vi "Day 11.vi"() -> ()   [LabVIEW 2021]
uses:
  <vilib>/Utility/file.llb/Read Delimited Spreadsheet (string).vi
panel:
  out "Input":i32[][](array[numeric])
  out "Part 2":i32
  out "Part 1":i32
  in  "Input File":enum32{"example input", "input"}(radio)
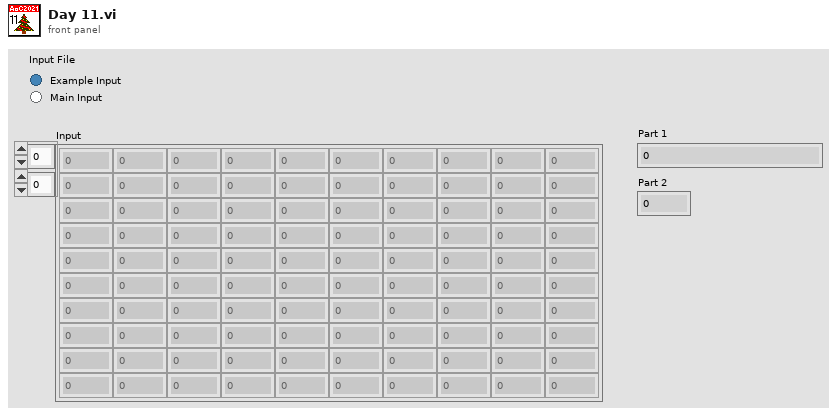
[diagram p1: front panel]
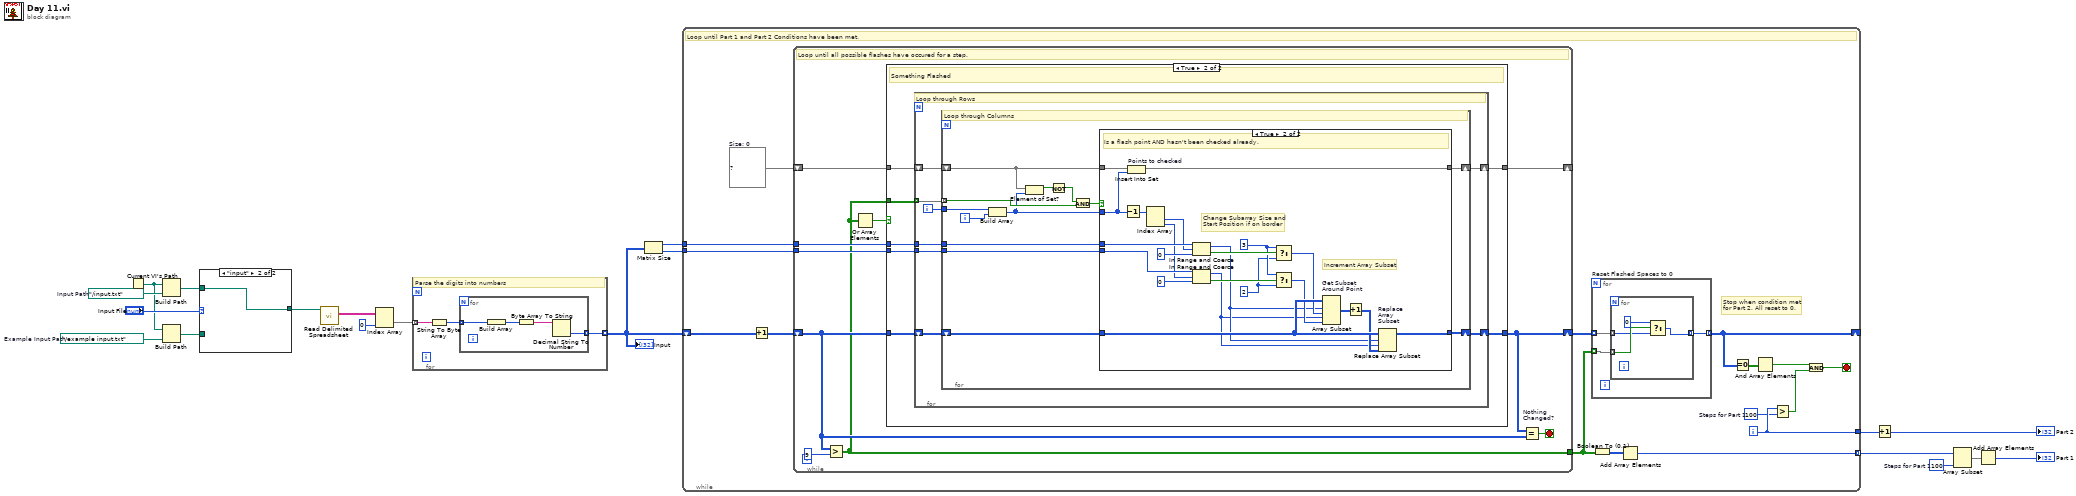
[diagram p0: block diagram]
diagram:
  w2 = 100  # Steps for Part 1
  w18 = path "../example input.txt"  # Example Input Path
  w19 = path "../input.txt"  # Input Path
  n1 = Current VI's Path() -> (path=w13:path)
  n2 = Build Path(base path=w13, name or relative path=w19) -> (appended path=w16:path)
  n3 = Build Path(base path=w13, name or relative path=w18) -> (appended path=w15:path)
  n4 = case shown="\"input\"" "Input File" {
    tunnel: w16 -> [_ w21]
    tunnel: w15 -> [w20 _]
    tunnel: [w20 w21] -> w14
    frame "example input" {
    }
    frame "input" {
    }
  }
  n5 = call-poly <vilib>:"Read Delimited Spreadsheet.vi"("file path (dialog if empty)"=w14) -> ("all rows"=w12:string[][])  [unwired: 9 in, 5 out]
  n6 = Index Array(array=w12, index (col)=0 ("disabled index (col)")) -> (element=w10:string[])  [unwired: 1 in]
  n7 = for {
    tunnel: w10 -> [w24] mode=indexing
    tunnel: [w22] -> w9 mode=indexing
    # "Parse the digits into numbers"
    n8 = String To Byte Array(string=w24) -> (unsigned byte array=w23:u8[])
    n9 = for {
      tunnel: w23 -> [w28] mode=indexing
      tunnel: [w25] -> w22 mode=indexing
      n10 = Build Array(w28) -> (w27:u8[])
      n11 = Byte Array To String(unsigned byte array=w27) -> (string=w26:string)
      n12 = Decimal String To Number(string=w26) -> (number=w25:i32)  [unwired: 2 in, 1 out]
    }
  }
  "Input" <- w9
  n13 = Matrix Size(0:w9) -> (1:w8:i32, 2:w7:i32)
  n14 = while {
    shift-right: [w38] -> _
    shift-left: w9 -> [w44]
    tunnel: w8 -> [w41]
    tunnel: w7 -> [w40]
    tunnel: [w33] -> w3 mode=indexing
    tunnel: [w31] -> w4
    i -> [w31]
    stop <- w32 stop-if-true
    w30 = 100  # Steps for Part 1
    w42 = set{i32[]} {}  # Size: 0
    # "Stop when condition met\nfor Part 2. All reset to 0."
    # "Loop until Part 1 and Part 2 Conditions have been met."
    n15 = Increment(x=w44) -> (x+1=w43:i32[][])
    n16 = while {
      shift-right: [w50] -> _
      shift-left: w42 -> [w53]
      tunnel: w41 -> [w52]
      tunnel: w40 -> [w51]
      shift-right: [w49] -> w39
      shift-left: w43 -> [w48]
      tunnel: [w45] -> w34
      stop <- w47 stop-if-true
      # "Loop until all possible flashes have occured for a step."
      n17 = Greater?(x=w48, y=9) -> (0:w45:bool[][])
      n18 = Or Array Elements(Boolean array=w45) -> (logical OR=w46:bool)
      n19 = case shown="True" w46 {
        tunnel: w53 -> [w56 w63]
        tunnel: w52 -> [_ w62]
        tunnel: w51 -> [_ w61]
        tunnel: [w56 w60] -> w50
        tunnel: [w55 w59] -> w49
        tunnel: w48 -> [w55 w58]
        tunnel: w45 -> [_ w57]
        frame False {
          # "Nothing Flashed"
        }
        frame True {
          # "Something Flashed"
          n20 = for {
            tunnel: w57 -> [w71] mode=indexing
            shift-right: [w68] -> w60
            shift-left: w63 -> [w69]
            shift-right: [w64] -> w59
            shift-left: w58 -> [w67]
            tunnel: w62 -> [w66]
            tunnel: w61 -> [w65]
            i -> [w70]
            # "Loop through Rows"
            n21 = for {
              tunnel: w71 -> [w84] mode=indexing
              tunnel: w70 -> [w83]
              shift-right: [w72] -> w68
              shift-left: w69 -> [w73]
              shift-right: [w74] -> w64
              shift-left: w67 -> [w77]
              tunnel: w66 -> [w76]
              tunnel: w65 -> [w75]
              i -> [w82]
              # "Loop through Columns"
              n22 = Build Array(w83, w82) -> (w81:i32[])
              n23 = Element of Set?(10:w81, 11:w73) -> (3:w79:bool)
              n24 = Not(x=w79) -> (.not. x?=w78:bool)
              n25 = And(x=w78, y=w84) -> (x .and. y?=w80:bool)
              n26 = case shown="True" w80 {
                tunnel: w81 -> [_ w108]
                tunnel: w77 -> [w86 w99]
                tunnel: w76 -> [_ w106]
                tunnel: w75 -> [_ w102]
                tunnel: [w86 w97] -> w74
                tunnel: w73 -> [w85 w94]
                tunnel: [w85 w93] -> w72
                frame False {
                }
                frame True {
                  w91 = 2
                  w92 = 3
                  # "Increment Array Subset"
                  # "Change Subarray Size and \nStart Position if on border"
                  # "Is a flash point AND hasn't been checked already."
                  n27 = Decrement(x=w108) -> (x-1=w107:i32[])
                  n28 = Insert Into Set "Points to checked"(10:w108, 11:w94) -> (3:w93:set{i32[]})  [unwired: 1 out]
                  n29 = Index Array(array=w107) -> (element #1=w90:i32, element #2=w88:i32)  [unwired: 2 in]
                  n30 = In Range and Coerce(upper limit=w106, x=w90, lower limit=0) -> (coerced(x)=w89:i32, In Range?=w104:bool)
                  n31 = In Range and Coerce(upper limit=w102, x=w88, lower limit=0) -> (coerced(x)=w87:i32, In Range?=w103:bool)
                  n32 = Select(t=w92, s=w104, f=w91) -> (s? t:f=w96:i32)
                  n33 = Select(t=w92, s=w103, f=w91) -> (s? t:f=w95:i32)
                  n34 = Array Subset "Get Subset\nAround Point"(array=w99, index (row)=w89, length (row)=w96, index (col)=w87, length (col)=w95) -> (w100:i32[][])
                  n35 = Increment(x=w100) -> (x+1=w98:i32[][])
                  n36 = Replace Array Subset "Replace\nArray\nSubset"(array=w99, new element=w98, index (row)=w89, index (col)=w87) -> (w97:i32[][])
                }
              }
            }
          }
        }
      }
      n37 = Equal? "Nothing\nChanged?"(x=w49, y=w48) -> (x = y?=w47:bool)
    }
    n38 = for "Reset Flashed Spaces to 0" {
      tunnel: w34 -> [w110] mode=indexing
      tunnel: w39 -> [w111] mode=indexing
      tunnel: [w109] -> w38 mode=indexing
      n39 = for {
        tunnel: w111 -> [w114] mode=indexing
        tunnel: w110 -> [w115] mode=indexing
        tunnel: [w112] -> w109 mode=indexing
        n40 = Select(t=0, s=w115, f=w114) -> (s? t:f=w112:i32)
      }
    }
    n41 = Boolean To (0,1)(Boolean=w34) -> (0, 1=w35:i16[][])
    n42 = Add Array Elements(numeric array=w35) -> (sum=w33:i16)
    n43 = Equal To 0?(x=w38) -> (x = 0?=w37:bool[][])
    n44 = And Array Elements(Boolean array=w37) -> (logical AND=w36:bool)
    n45 = Greater?(x=w31, y=w30) -> (0:w29:bool)
    n46 = And(x=w36, y=w29) -> (x .and. y?=w32:bool)
  }
  n47 = Increment(x=w4) -> (x+1=→"Part 2":i32)
  n48 = Array Subset(array=w3, length=w2) -> (w1:i16[])  [unwired: 1 in]
  n49 = Add Array Elements(numeric array=w1) -> (sum=→"Part 1":i16)
